vi "Load_Recipe.vi"(8 "error in (no error)":errorcluster, 10 "Recipe Name":string, 11 "Recipe Dir":path) -> (0 "error out":errorcluster, 3 "Recipe":T1)   [LabVIEW 2018]
uses:
  Recipe.ctl
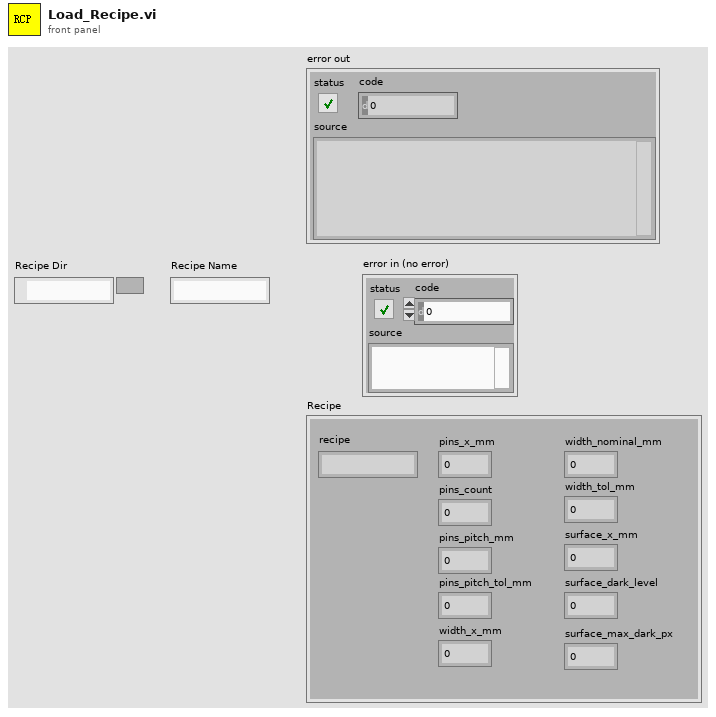
[diagram p1: front panel]
types:
  T1 = typedef "Recipe.ctl" = cluster{"recipe":string, "pins_x_mm":dbl, "pins_count":i32, "pins_pitch_mm":dbl, "width_x_mm":dbl, "width_nominal_mm":dbl, "surface_max_dark_px":i32, "surface_dark_level":dbl, "surface_x_mm":dbl, "width_tol_mm":dbl, "pins_pitch_tol_mm":dbl}
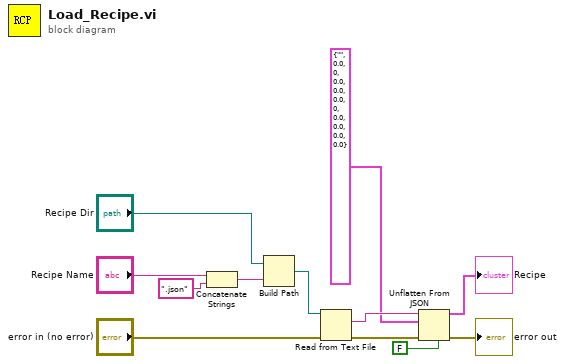
[diagram p0: block diagram]
diagram:
  n1 = Concatenate Strings("Recipe Name", ".json" ("string")) -> (w9:string)
  n2 = Build Path(base path="Recipe Dir", name or relative path=w9) -> (appended path=w8:path)
  n3 = Read from Text File(file (use dialog)=w8, error in="error in (no error)") -> (text=w6:string, error out=w4:errorcluster)  [unwired: 2 in, 2 out]
  n4 = Unflatten From JSON(JSON string=w6, type and defaults=T1 {"recipe"="", "pins_x_mm"=0.0, "pins_count"=0, "pins_pitch_mm"=0.0, "width_x_mm"=0.0, "width_nominal_mm"=0.0, "surface_max_dark_px"=0, "surface_dark_level"=0.0, "surface_x_mm"=0.0, "width_tol_mm"=0.0, "pins_pitch_tol_mm"=0.0} ("Recipe"), strict validation? (F)=FALSE, error in (no error)=w4) -> (value=→"Recipe":T1, error out=→"error out":errorcluster)  [unwired: 3 in]
